vi "A_Loop_Inverted.vi"(0 "Numeric":i32, 1 "x":dbl, 5 "instrument handle out":refnum<k15>, 7 "Numeric 2":i32, 9 "Numeric 3":i32, 11 "Numeric 4":dbl, 12 "Tset setting":dbl, 14 "N per point":i32) -> (4 "output array":string[](array[string]), 6 "output array 2":string[](array[string]), 10 "Array 3":string[](array[string]))   [LabVIEW 2025]
panel:
  out "error out":errorcluster
  out "Array 2":string[](array[string])
  out "Array":string[](array[string])
  out "Slide":dbl(slide) scale=0.1..100.0
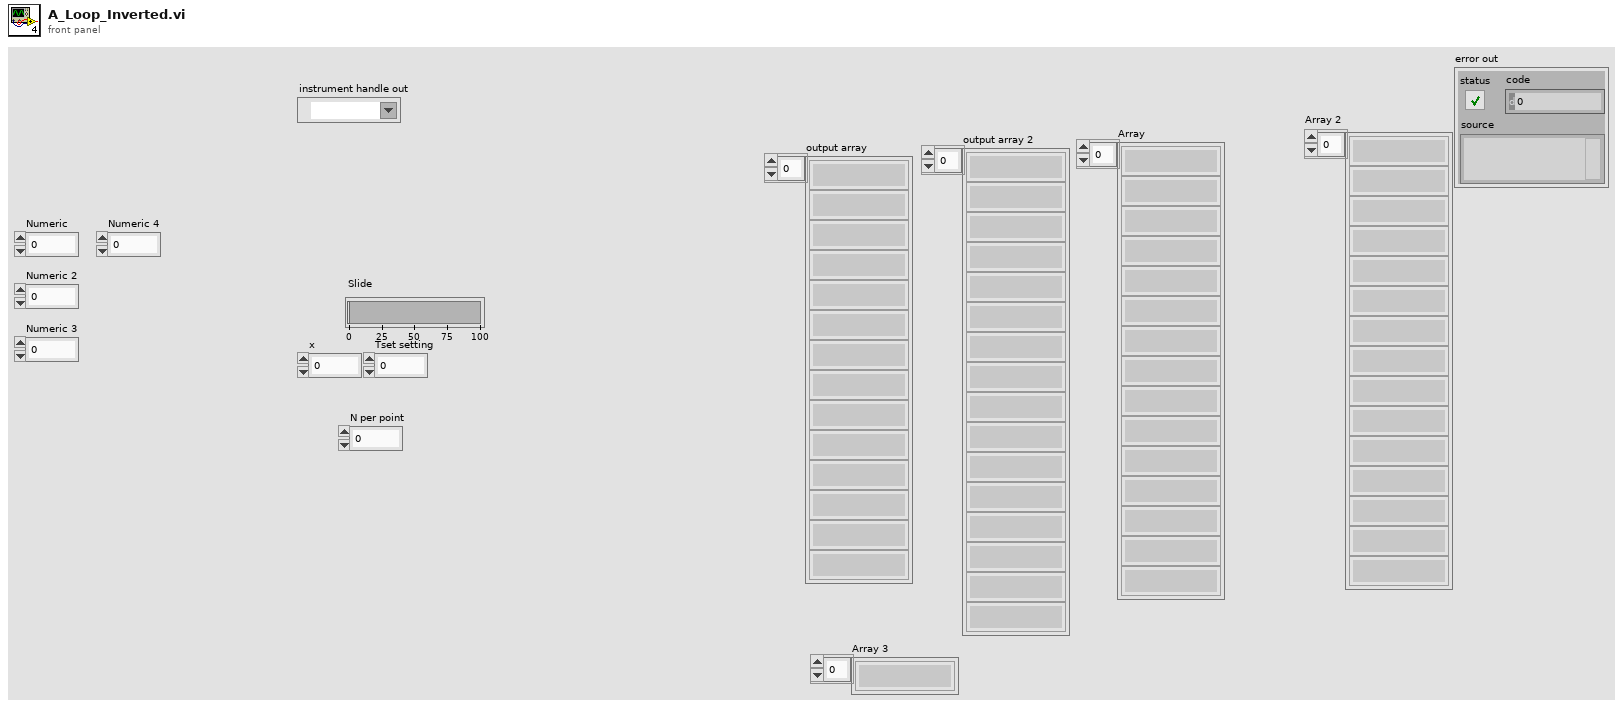
[diagram p1: front panel]
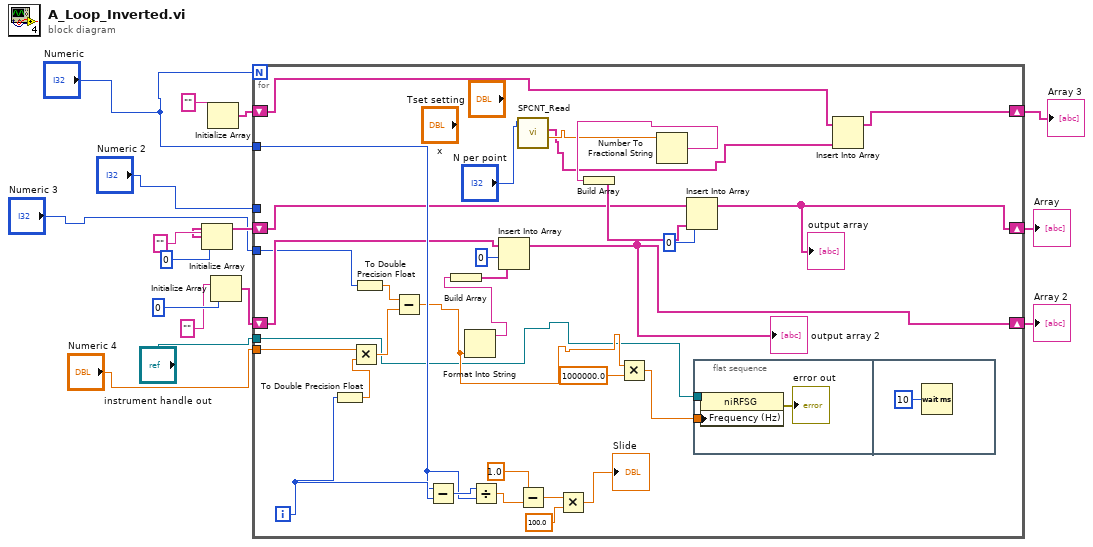
[diagram p0: block diagram]
diagram:
  n1 = Initialize Array("", 0 ("dimension size")) -> (w12:string[])
  n2 = Initialize Array("") -> (w3:string[])  [unwired: 1 in]
  n3 = Initialize Array("", 0 ("dimension size")) -> (w11:string[])
  n4 = for {
    N: "Numeric" -> [_]
    tunnel: "Numeric 4" -> [w48]
    tunnel: "Numeric 2" -> [_]
    tunnel: "Numeric" -> [w39]
    tunnel: "Numeric 3" -> [w26]
    shift-right: [w28] -> w10
    shift-left: w12 -> [w30]
    shift-right: [w31] -> w9
    shift-left: w11 -> [w29]
    shift-right: [w24] -> w2
    shift-left: w3 -> [w25]
    tunnel: "instrument handle out" -> [w18]
    i -> [w41]
    n5 = To Double Precision Float(number=w41) -> (double precision float=w47:dbl)
    n6 = Multiply(x=w48, y=w47) -> (x*y=w32:dbl)
    n7 = To Double Precision Float(number=w26) -> (double precision float=w33:dbl)
    n8 = Subtract(x=w33, y=w32) -> (x-y=w19:dbl)
    n9 = Subtract(x=w39, y=w41) -> (x-y=w40:i32)
    n10 = Format Into String(w19) -> (resulting string=w42:string)  [unwired: 3 in, 1 out]
    n11 = Build Array(w42) -> (w46:string[])
    n12 = Divide(x=w40, y=w39) -> (x/y=w37:dbl)
    n13 = Insert Into Array "Insert Into Array"(array=w29, index=0 ("index (row)"), new element=w46) -> (w31:string[])
    "output array 2" <- w31
    n14 = call "SPCNT_Read.vi"("N per point"="N per point") -> ("x/y"=w22:dbl, "Array"=w21:string[])  [unwired: 9 in]
    n15 = Subtract(x=1.0, y=w37) -> (x-y=w36:dbl)
    n16 = Multiply(x=w36, y=100.0) -> (x*y=→"Slide":dbl)
    n17 = Multiply(x=w19, y=1000000.0) -> (x*y=w17:dbl)
    n18 = Number To Fractional String(number=w22) -> (F-format string=w34:string)  [unwired: 3 in]
    n19 = Build Array(w34) -> (w44:string[])
    n20 = Insert Into Array "Insert Into Array"(array=w30, index=0, new element=w44) -> (w28:string[])
    "output array" <- w28
    n21 = flat-sequence {
      tunnel: w18 -> [w51]
      tunnel: w17 -> [w50]
      frame #0 {
        n22 = property class="niRFSG"(reference=w51, "Frequency (Hz)"=w50) -> (error out=→"error out":errorcluster)  [unwired: 1 in, 1 out]
      }
      frame #1 {
        n23 = Wait (ms)(milliseconds to wait=u32 10) -> ()  [unwired: 1 out]
      }
    }
    n24 = Insert Into Array(array=w25, new element=w21) -> (w24:string[])  [unwired: 1 in]
  }
  "Array" <- w10
  "Array 2" <- w9
  "Array 3" <- w2
